vi "ControlSolenoids.vi"(0 "Joystick Refnum Name":string) -> ()   [LabVIEW 2014]
uses:
  <vilib>/Rock Robotics/WPI/Relay/WPI_RelayValue.ctl
  <vilib>/Rock Robotics/WPI/Joystick/WPI_JoystickGetSetRefNum.vi
  <vilib>/Rock Robotics/Network Tables/SD Write Boolean Array.vi
  <vilib>/Rock Robotics/Network Tables/SD Write Numeric Array.vi
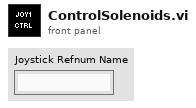
[diagram p1: front panel]
types:
  T1 = typedef "WPI_RelayValue.ctl" = enum16{"Off", "On", "Forward", "Reverse"}
  T2 = typedef "WPI_JoystickDevRef.ctl" = cluster{"Device":T3}
  T3 = typedef "WPI_JoystickDeviceEnum.ctl" = enum16{"USB 0", "USB 1", "USB 2", "USB 3", "USB 4", "USB 5"}
  T4 = typedef "WPI_RelayDevRef.ctl" = cluster{"DevStatus":errorcluster, "Relay Channel":T5, "Controller":T6, "Relay Direction":T7}
  T5 = typedef "FPGA_DIORelayChannel.ctl" = enum8{"Relay 0", "Relay 1", "Relay 2", "Relay 3", "Invalid"}
  T6 = typedef "FPGA_TypedefDigitalModule.ctl" = enum16{"Controller 1"}
  T7 = typedef "WPI_RelayDirection.ctl" = enum16{"Both directions", "Forward only", "Reverse only"}
  T8 = typedef "WPI_DigitalInputDevRef.ctl" = cluster{"DevStatus":errorcluster, "DIO Channel":T9, "Controller":T6}
  T9 = typedef "FPGA_DIOChannel.ctl" = enum8{"DIO 0", "DIO 1", "DIO 2", "DIO 3", "DIO 4", "DIO 5", "DIO 6", "DIO 7", "DIO 8", "DIO 9", "DIO MXP 0", "DIO MXP 1", "DIO MXP 2", "DIO MXP 3", "DIO MXP 4", "DIO MXP 5", "DIO MXP 6", "DIO MXP 7", "DIO MXP 8", "DIO MXP 9", "DIO MXP 10", "DIO MXP 11", "DIO MXP 12", "DIO MXP 13", "DIO MXP 14", "DIO MXP 15", "Invalid"}
  T10 = typedef "WPI_MotorControlDeviceRef.ctl" = cluster{"DeviceStatus":errorcluster, "Type":T11, "PWM":cluster{"Controller":T6, "PWM Channel":T12, "DeadBand":T13}, "CAN":cluster{"Device Number":u8, "Control Mode":T14, "Semaphore":T15, "Max Vout":dbl, "TalonSRX Control Mode":T16}, "Invert":bool, "TransformRef":T17, "InvTransformRef":T17}
  T11 = typedef "WPI_MotorControlType.ctl" = enum16{"PWM", "CAN", "CANTalonSRX"}
  T12 = typedef "FPGA_DIOPWMChannel.ctl" = enum8{"PWM 0", "PWM 1", "PWM 2", "PWM 3", "PWM 4", "PWM 5", "PWM 6", "PWM 7", "PWM 8", "PWM 9", "PWM MXP 0", "PWM MXP 1", "PWM MXP 2", "PWM MXP 3", "PWM MXP 4", "PWM MXP 5", "PWM MXP 6", "PWM MXP 7", "PWM MXP 8", "PWM MXP 9", "Invalid"}
  T13 = typedef "WPI_PWMDeadband.ctl" = cluster{"Name":string, "maxPositivePwm":i32, "minPositivePwm":i32, "centerPwm":i32, "maxNegativePwm":i32, "minNegativePwm":i32, "angularRange":u16}
  T14 = typedef "WPI_CANJaguar_ControlMode.ctl" = enum8{"Percent VBus", "Current", "Speed", "Position", "Voltage"}
  T15 = typedef "Semaphore RefNum" = refnum<k1>
  T16 = typedef "WPI_CANTalonSRX_APIControlMode.ctl" = enum8{"Percent VBus", "Speed", "Position", "Slave", "Unchanged / Invalid"}
  T17 = typedef "WPI_PWMTransform_ConPane.ctl" = refnum<vi>
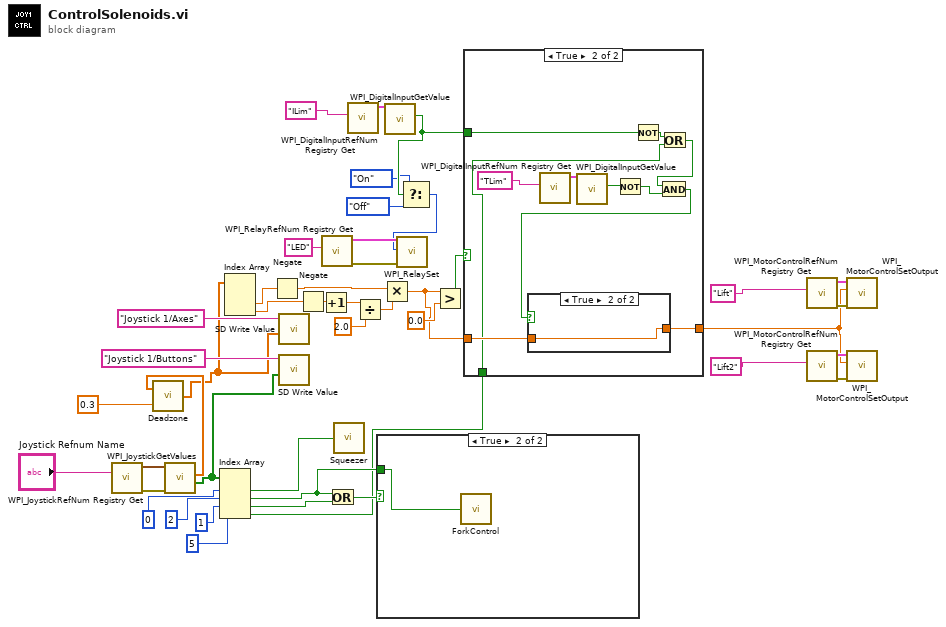
[diagram p0: block diagram]
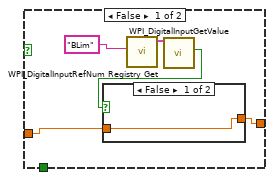
[diagram p3: hidden frame]
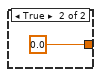
[diagram p4: hidden frame]
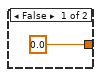
[diagram p5: hidden frame]
diagram:
  n1 = call <vilib>:"WPI_JoystickRefNum Registry Get.vi"("refnum name"="Joystick Refnum Name") -> ("error out"=w43:errorcluster, "JoystickDevRef"=w42:T2)  [unwired: 9 in]
  n2 = call <vilib>:"WPI_JoystickGetValues.vi"("error in (no error)"=w43, "JoystickDevRef"=w42) -> ("Buttons"=w34:bool[], "Axes"=w29:dbl[])  [unwired: 5 in, 3 out]
  n3 = call "Deadzone.vi"("Deadzone"=0.3, "Joystick Axes In"=w29) -> ("Joystick Axes Out"=w28:dbl[])
  n4 = Index Array(array=w34, index #1=0, index #2=2, index #3=1, index #4=5 ("index")) -> (element #1=w20:bool, element #2=w37:bool, element #3=w38:bool, element #4=w14:bool)
  n5 = Index Array(array=w28) -> (element #2=w27:dbl, element #3=w21:dbl)  [unwired: 3 in, 1 out]
  n6 = Negate(x=w27) -> (-x=w23:dbl)
  n7 = call-poly <vilib>:"SD Write Value.vi"("Numeric Array"=w28, "Name"="Joystick 1/Axes") -> ()  [unwired: 8 in, 2 out]
  n8 = call-poly <vilib>:"SD Write Value.vi"("Boolean Array"=w34, "Name"="Joystick 1/Buttons") -> ()  [unwired: 8 in, 2 out]
  n9 = Negate(x=w21) -> (-x=w22:dbl)
  n10 = Increment(x=w22) -> (x+1=w26:dbl)
  n11 = call <vilib>:"WPI_RelayRefNum Registry Get.vi"("refnum name"="LED") -> ("error out"=w11:errorcluster, "RelayDevRef"=w10:T4)  [unwired: 9 in]
  n12 = Or(x=w37, y=w38) -> (x .or. y?=w15:bool)
  n13 = call "Squeezer.vi"("Direction"=w20) -> ()
  n14 = call <vilib>:"WPI_DigitalInputRefNum Registry Get.vi"("refnum name"="ILim") -> ("DigitalInputDevRef"=w13:T8)  [unwired: 9 in, 1 out]
  n15 = Divide(x=w26, y=2.0) -> (x/y=w24:dbl)
  n16 = case shown="True" w15 {
    tunnel: w37 -> [_ w45]
    frame False {
    }
    frame True {
      n17 = call "ForkControl.vi"("Direction"=w45) -> ()
    }
  }
  n18 = Multiply(x=w23, y=w24) -> (x*y=w16:dbl)
  n19 = call <vilib>:"WPI_DigitalInputGetValue.vi"("DigitalInputDevRef"=w13) -> ("Value"=w7:bool)  [unwired: 8 in, 2 out]
  n20 = Select(t=WPI_RelayValue."On" ("RelayValue"), s=w7, f=WPI_RelayValue."Off" ("RelayValue")) -> (s? t:f=w5:T1)
  n21 = call <vilib>:"WPI_RelaySet.vi"("error in (no error)"=w11, "RelayValue"=w5, "RelayDevRef"=w10) -> ()  [unwired: 7 in, 2 out]
  n22 = Greater?(x=w16, y=0.0) -> (0:w17:bool)
  n23 = case shown="True" w17 {
    tunnel: [w46 w61] -> w1
    tunnel: w16 -> [w47 w60]
    tunnel: w14 -> [_ w55]
    tunnel: w7 -> [_ w53]
    frame False {
      n24 = call <vilib>:"WPI_DigitalInputRefNum Registry Get.vi"("refnum name"="BLim") -> ("DigitalInputDevRef"=w50:T8)  [unwired: 9 in, 1 out]
      n25 = call <vilib>:"WPI_DigitalInputGetValue.vi"("DigitalInputDevRef"=w50) -> ("Value"=w48:bool)  [unwired: 8 in, 2 out]
      n26 = case shown="False" w48 {
        tunnel: [w51 0.0] -> w46
        tunnel: w47 -> [w51 _]
        frame False {
        }
        frame True {
        }
      }
    }
    frame True {
      n27 = call <vilib>:"WPI_DigitalInputRefNum Registry Get.vi"("refnum name"="TLim") -> ("DigitalInputDevRef"=w63:T8)  [unwired: 9 in, 1 out]
      n28 = call <vilib>:"WPI_DigitalInputGetValue.vi"("DigitalInputDevRef"=w63) -> ("Value"=w58:bool)  [unwired: 8 in, 2 out]
      n29 = Not(x=w58) -> (.not. x?=w57:bool)
      n30 = Not(x=w53) -> (.not. x?=w56:bool)
      n31 = Or(x=w56, y=w55) -> (x .or. y?=w54:bool)
      n32 = And(x=w54, y=w57) -> (x .and. y?=w59:bool)
      n33 = case shown="True" w59 {
        tunnel: [0.0 w65] -> w61
        tunnel: w60 -> [_ w65]
        frame False {
        }
        frame True {
        }
      }
    }
  }
  n34 = call <vilib>:"WPI_MotorControlRefNum Registry Get.vi"("refnum name"="Lift") -> ("error out"=w32:errorcluster, "MotorControlDevRef"=w31:T10)  [unwired: 9 in]
  n35 = call <vilib>:"WPI_MotorControlRefNum Registry Get.vi"("refnum name"="Lift2") -> ("error out"=w3:errorcluster, "MotorControlDevRef"=w2:T10)  [unwired: 9 in]
  n36 = call <vilib>:"WPI_MotorControlSetOutput.vi"("error in (no error)"=w32, "Output"=w1, "MotorControlDevRef"=w31) -> ()  [unwired: 6 in, 3 out]
  n37 = call <vilib>:"WPI_MotorControlSetOutput.vi"("error in (no error)"=w3, "Output"=w1, "MotorControlDevRef"=w2) -> ()  [unwired: 6 in, 3 out]
